vi "Display.vi"(8 "error in":errorcluster, 11 "Plain - Two Button in":refnum<class "Plain - Two Button.lvclass">) -> (0 "error out":errorcluster, 3 "Plain - Two Button out":refnum<class "Plain - Two Button.lvclass">)   [LabVIEW 2021, in "Pop-Up.lvlib" / "Plain - Two Button.lvclass"]
doc: "This is the override method required for each child of the pop up class. It is the pop up that will display to the user.\n\nTo extend this function, create a child class of the pop up class. Then create an override method for this VI. <b>Display.vi</b> is a protected function, therefore it cannot be called in a main application. This VI must be called by a caller function. See one of the standard pop-ups for a setup example.\n\n<b>Code Developed By:</b> +\nDaniel Coons +\nhttps://github.com/danielcoons/tsc-pop-up"
uses:
  Plain - Two Button.lvclass
  C:/Development/Open Source/tsc-pop-up/Popup/Popup.lvclass
  C:/Development/Open Source/tsc-pop-up/Plain/Plain Parent.lvclass
  Popup/Popup.lvclass/Popup.ctl
  Plain Parent.lvclass/Plain Parent.ctl
  Popup/Data Member Access/Read Theme.vi
  Get Transparent buttons.vi
  Get Dialog Title.vi
  Get Action 1 Text.vi
  Get Action 2 Text.vi
  Theme/Theme.lvclass
  Plain - Two Button.lvclass/Plain - Two Button.ctl
  Popup/Popup.lvclass
  user32.dll
panel:
  in  "action 2":bool
  out "dialog title":string
  out "message":string
  in  "action 1":bool
  # "This VI displays the popup"
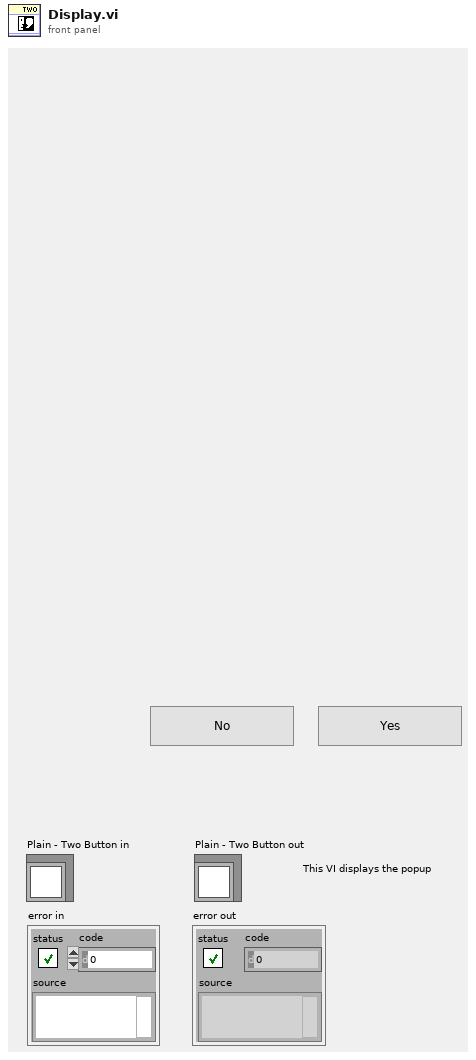
[diagram p1: front panel]
types:
  T1 = typedef "LVRectTypeDef.ctl" = cluster{"Left":i16, "Top":i16, "Right":i16, "Bottom":i16}
  T2 = typedef "LVPointTypeDef.ctl" = cluster{"Horizontal":i16, "Vertical":i16}
  T3 = typedef "LVPoint32TypeDef.ctl" = cluster{"Horizontal":i32, "Vertical":i32}
  T4 = typedef "LVPositionTypeDef.ctl" = cluster{"Left":i32, "Top":i32}
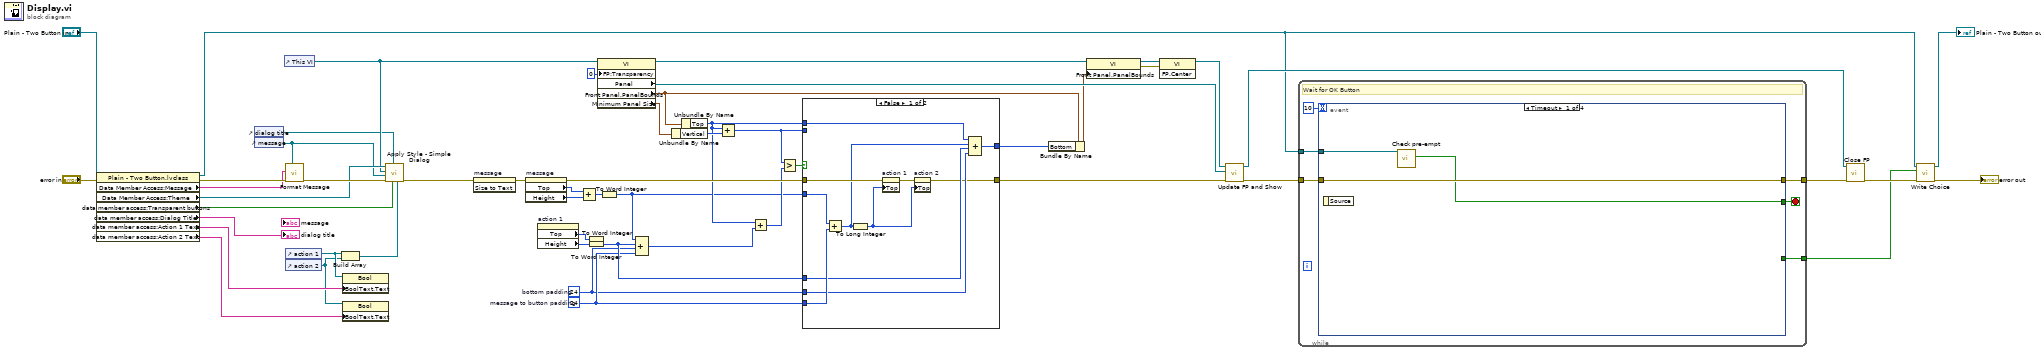
[diagram p0: block diagram]
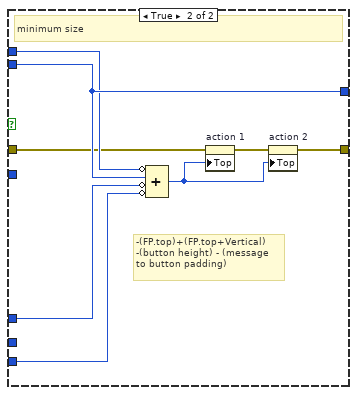
[diagram p2: hidden frame]
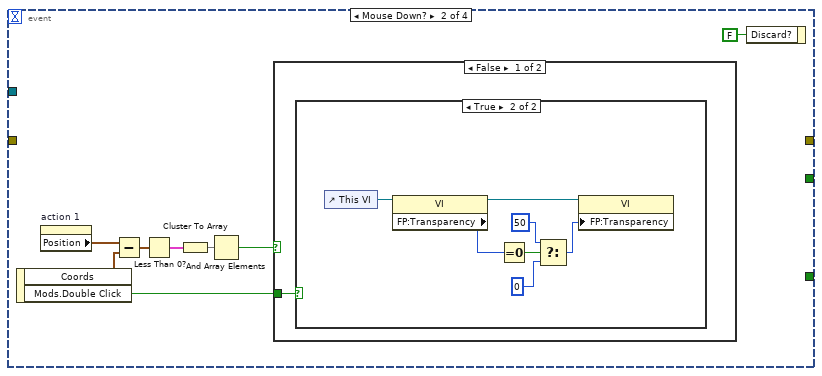
[diagram p3: hidden frame]
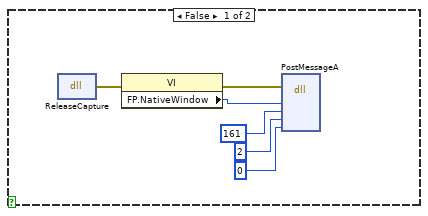
[diagram p4: hidden frame]
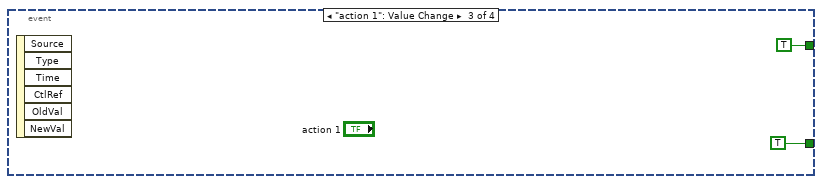
[diagram p6: hidden frame]
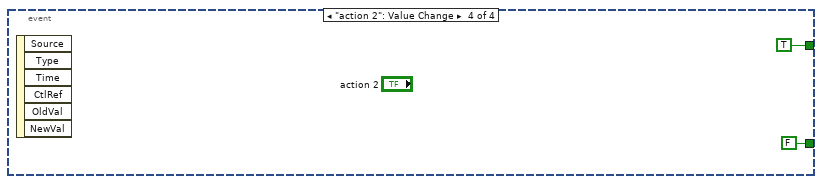
[diagram p7: hidden frame]
diagram:
  w28 = i16 24  # message to button padding
  w26 = i16 24  # bottom padding
  n1 = property class="Plain - Two Button.lvclass"(reference="Plain - Two Button in", error in="error in") -> (reference out=w8:refnum<class "Plain - Two Button.lvclass">, error out=w49:errorcluster, "Data Member Access:Message"=w47:string, "Data Member Access:Theme"=w20:refnum<class "Theme.lvclass">, "data member access:Transparent buttons"=w1:bool, "data member access:Dialog Title"=→"dialog title":string, "data member access:Action 1 Text"=w15:string, "data member access:Action 2 Text"=w10:string)
  n2 = control-ref of="dialog title"() -> (w5:refnum<vi>)
  n3 = control-ref of="message"() -> (w4:refnum<vi>)
  n4 = control-ref of="This VI"() -> (w19:refnum<vi>)
  n5 = call "Format Message.vi"("formatted string"=w4, "error in"=w49, "String Input"=w47) -> ("error out"=w22:errorcluster)  [unwired: 7 in, 1 out]
  n6 = control-ref of="action 1"() -> (w16:refnum<vi>)
  n7 = control-ref of="action 2"() -> (w11:refnum<vi>)
  n8 = Build Array(w16, w11) -> (w18:refnum<vi>[])
  n9 = property class="Bool"(reference=w16, "BoolText.Text"=w15) -> ()  [unwired: 1 in, 2 out]
  n10 = property class="Bool"(reference=w11, "BoolText.Text"=w10) -> ()  [unwired: 1 in, 2 out]
  n11 = call "Apply Style - Simple Dialog.vi"("button refs"=w18, "keep transparent buttons?"=w1, "title ref"=w5, "error in"=w22, "message ref"=w4, "pop up ref"=w19, "Theme in"=w20) -> ("error out"=w21:errorcluster)  [unwired: 3 in, 1 out]
  n12 = invoke on="message" class="Str" method="Size to Text"(error in=w21) -> (error out=w48:errorcluster)  [unwired: 2 in, 2 out]
  n13 = property on="message" class="Str"(error in=w48) -> (error out=w31:errorcluster, "Top"=w42:i32, "Height"=w41:u32)  [unwired: 1 in, 1 out]
  n14 = property on="action 1" class="Bool"() -> ("Top"=w44:i32, "Height"=w43:u32)  [unwired: 2 in, 2 out]
  n15 = Add(x=w42, y=w41) -> (x+y=w40:u32)
  n16 = To Word Integer(number=w44) -> ()  [unwired: 1 out]
  n17 = To Word Integer(number=w43) -> (16bit integer=w29:i16)
  n18 = property class="VI"(reference=w19, "FP:Transparency"=u8 0 ("Front Panel Window:Transparency")) -> (reference out=w46:refnum<vi>, "Panel"=w45:refnum<vi>, "Front Panel.PanelBounds"=w36:T1, "Minimum Panel Size"=w39:T2)  [unwired: 1 in, 1 out]
  n19 = To Word Integer(number=w40) -> (16bit integer=w3:i16)
  n20 = Compound Arithmetic op=ADD(w3, w29, w26, w28) -> (w2:i16)
  n21 = Unbundle By Name(w39) -> ("Vertical"=w38:i16)
  n22 = Unbundle By Name(w36) -> ("Top"=w23:i16)
  n23 = Add(x=w23, y=w38) -> (x+y=w24:i16)
  n24 = Add(x=w23, y=w2) -> (x+y=w25:i16)
  n25 = Greater?(x=w24, y=w25) -> (0:w32:bool)
  n26 = case shown="False" w32 {
    tunnel: [w63 w72] -> w27
    tunnel: w24 -> [_ w72]
    tunnel: w3 -> [w64 _]
    tunnel: w23 -> [w57 w71]
    tunnel: w31 -> [w62 w70]
    tunnel: [w55 w66] -> w30
    tunnel: w29 -> [w59 w69]
    tunnel: w28 -> [w61 w68]
    tunnel: w26 -> [w60 _]
    frame False {
      n27 = Add(x=w64, y=w61) -> (x+y=w58:i16)
      n28 = To Long Integer(number=w58) -> (32bit integer=w54:i32)
      n29 = property on="action 1" class="Bool"(error in=w62, "Top"=w54) -> (error out=w56:errorcluster)  [unwired: 1 in, 1 out]
      n30 = property on="action 2" class="Bool"(error in=w56, "Top"=w54) -> (error out=w55:errorcluster)  [unwired: 1 in, 1 out]
      n31 = Compound Arithmetic op=ADD(w57, w58, w59, w60) -> (w63:i16)
    }
    frame True {
      # "-(FP.top)+(FP.top+Vertical)\n-(button height) - (message\nto button padding)"
      # "minimum size"
      n32 = Compound Arithmetic op=ADD(invert w71, w72, invert w69, invert w68) -> (w65:i16)
      n33 = property on="action 1" class="Bool"(error in=w70, "Top"=w65) -> (error out=w67:errorcluster)  [unwired: 1 in, 1 out]
      n34 = property on="action 2" class="Bool"(error in=w67, "Top"=w65) -> (error out=w66:errorcluster)  [unwired: 1 in, 1 out]
    }
  }
  n35 = Bundle By Name(cluster=w36, "Bottom"=w27) -> (w33:T1)
  n36 = property class="VI"(reference=w46, "Front Panel.PanelBounds"=w33) -> (reference out=w37:refnum<vi>, error out=w34:errorcluster)  [unwired: 1 in]
  n37 = invoke class="VI" method="FP.Center"(reference=w37, error in=w34) -> (reference out=w35:refnum<vi>)  [unwired: 1 in, 2 out]
  n38 = call "Update FP and Show.vi"("error in (no error)"=w30, "Panel Ref"=w45, "VI in"=w35) -> ("error out"=w52:errorcluster, "VI out"=w51:refnum<vi>)  [unwired: 7 in]
  n39 = while {
    tunnel: [w76] -> w53
    tunnel: w52 -> [w77]
    tunnel: w8 -> [w74]
    tunnel: [w73] -> w7
    stop <- w78 stop-if-true
    # "Wait for OK Button"
    n40 = event shown="[0] Timeout" {
      selector: _ -> [_ _ _ _]
      dyn-events: _ -> [_ _ _ _]
      timeout: 10 -> [_ _ _ _]
      tunnel: [w79 _ TRUE ("Pre-empted?") TRUE ("Pre-empted?")] -> w78
      tunnel: w77 -> [w81 _ _ _]
      tunnel: [w81 _ _ _] -> w76
      tunnel: w74 -> [w80 _ _ _]
      tunnel: [_ _ TRUE FALSE] -> w73
      event Timeout {
        n41 = event-data() -> ()  [unwired: 1 in, 1 out]
        n42 = call "Check pre-empt.vi"("_Popup in"=w80) -> ("Pre-empted?"=w79:bool)  [unwired: 8 in, 2 out]
      }
      event Mouse Down? {
        n43 = event-data() -> ("Coords"=w83:T3, "Mods.Double Click"=w85:bool)  [unwired: 1 in]
        n44 = property on="action 1" class="Bool"() -> ("Position"=w84:T4)  [unwired: 2 in, 2 out]
        n45 = Subtract(x=w84, y=w83) -> (x-y=w86:T4)
        n46 = Less Than 0?(x=w86) -> (x < 0?=w87:cluster{"Left":bool, "Top":bool})
        n47 = Cluster To Array(cluster=w87) -> (array=w88:bool[])
        n48 = And Array Elements(Boolean array=w88) -> (logical AND=w89:bool)
        n49 = case shown="False" w89 {
          tunnel: w85 -> [w90 _]
          frame False {
            n50 = case shown="True" w90 {
              frame False {
                n51 = dll-call lib="user32.dll" fn="ReleaseCapture"() -> (error out=w94:errorcluster)  [unwired: 4 in, 1 out]
                n52 = property class="VI"(error in=w94) -> (error out=w95:errorcluster, "FP.NativeWindow"=w96:u64)  [unwired: 1 in, 1 out]
                n53 = dll-call lib="user32.dll" fn="PostMessageA"(error in=w95, "hWnd"=w96, "Msg"=161, "wParam"=2, "lParam"=0) -> ()  [unwired: 7 in, 2 out]
              }
              frame True {
                n54 = control-ref of="This VI"() -> (w103:refnum<vi>)
                n55 = property class="VI"(reference=w103) -> (reference out=w101:refnum<vi>, "FP:Transparency"=w102:u8)  [unwired: 1 in, 1 out]
                n56 = Equal To 0?(x=w102) -> (x = 0?=w100:bool)
                n57 = Select(t=u8 50, s=w100, f=u8 0) -> (s? t:f=w99:u8)
                n58 = property class="VI"(reference=w101, "FP:Transparency"=w99) -> ()  [unwired: 1 in, 2 out]
              }
            }
          }
          frame True {
          }
        }
        n59 = event-data("Discard?"=FALSE) -> ()  [unwired: 1 in, 1 out]
      }
      event "action 1": Value Change {
        n60 = event-data() -> ()  [unwired: 1 in, 6 out]
      }
      event "action 2": Value Change {
        n61 = event-data() -> ()  [unwired: 1 in, 6 out]
      }
    }
  }
  n62 = call "Close FP.vi"("error in (no error)"=w53, "VI in"=w51) -> ("error out"=w14:errorcluster)  [unwired: 9 in]
  n63 = call-dynamic "Write Choice.vi"("error in (no error)"=w14, "Choice"=w7, "_Popup in"=w8) -> ("error out"=→"error out":errorcluster, "_Popup out"=→"Plain - Two Button out":refnum<class "Plain - Two Button.lvclass">)  [unwired: 7 in]
